vi "write config ini data.vi"(8 "error in (no error)":errorcluster, 10 "data in":T2={"sections"=[], "key names"=[], "values"=[]}, 11 "Refnum in":T1) -> (0 "error out":errorcluster, 3 "Refnum out":T1)   [LabVIEW 2018, in "Config Files Management.lvlib"]
doc: "This function writes the complete data from the input cluster to a configuration .ini file, regardless of the number of sections or the number of keys in each section. The input is a cluster containing three string arrays: a 2-D array for the sections, where the first row stores the section names and the second row contains the number of keys in each section; a 1-D string array for the key names; and a 1-D string array for the corresponding values."
uses:
  Config Files Management.lvlib
  <vilib>/Utility/config.llb/NI_LVConfig.lvlib
  <vilib>/Utility/config.llb/Write Key (String).vi
  <vilib>/Utility/config.llb/Config Data RefNum.ctl
  config data--cluster.ctl
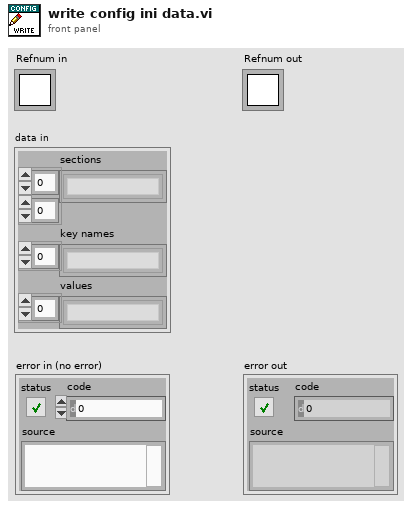
[diagram p1: front panel]
types:
  T1 = typedef "NI_LVConfig.lvlib/Config Data RefNum.ctl" = refnum<k1>
  T2 = typedef "Config Files Management.lvlib/config data--cluster.ctl" = cluster{"sections":string[][], "key names":string[], "values":string[]}
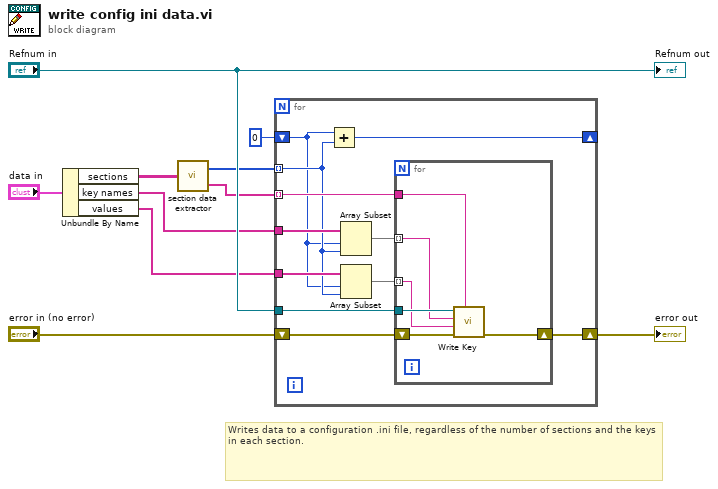
[diagram p0: block diagram]
diagram:
  # "Writes data to a configuration .ini file, regardless of the number of sections and the keys in each section."
  n1 = Unbundle By Name("data in") -> ("sections"=w6:string[][], "key names"=w8:string[], "values"=w7:string[])
  n2 = call "section data extractor.vi"("sections data"=w6) -> ("#keys per section"=w4:i32[], "sections"=w5:string[])  [unwired: 4 in]
  n3 = for {
    tunnel: w7 -> [w14]
    tunnel: w8 -> [w17]
    tunnel: "Refnum in" -> [w20]
    tunnel: w5 -> [w19] mode=indexing
    shift-right: [w18] -> w2
    shift-left: "error in (no error)" -> [w21]
    tunnel: w4 -> [w12] mode=indexing
    shift-right: [w15] -> _
    shift-left: 0 ("sector") -> [w11]
    n4 = Add(x=w11, y=w12) -> (x+y=w15:i32)
    n5 = Array Subset(array=w17, index=w11, length=w12) -> (w16:string[])
    n6 = Array Subset(array=w14, index=w11, length=w12) -> (w13:string[])
    n7 = for {
      tunnel: w20 -> [w27]
      shift-right: [w22] -> w18
      shift-left: w21 -> [w26]
      tunnel: w19 -> [w25]
      tunnel: w16 -> [w24] mode=indexing
      tunnel: w13 -> [w23] mode=indexing
      n8 = call-poly <vilib>:"Write Key.vi"("section"=w25, "error in (no error)"=w26, "value"=w23, "key"=w24, "refnum"=w27) -> ("error out"=w22:errorcluster)  [unwired: 4 in, 2 out]
    }
  }
  "error out" <- w2
  "Refnum out" <- "Refnum in"
